vi "HMI.vi"() -> ()   [LabVIEW 2018]
uses:
  <vilib>/Platform/TimedLoop/XDataNode/timing_clust.ctl
  <vilib>/Platform/TimedLoop/XDataNode/nitl_modes.ctl
  <vilib>/Platform/TimedLoop/XDataNode/wakeup.ctl
  <vilib>/Instr/_visa.llb/VISA Configure Serial Port (Instr).vi
  <vilib>/Utility/file.llb/Write Delimited Spreadsheet (DBL).vi
  <vilib>/platform/TimedLoop/XDataNode/XDataNode.xnode
  <vilib>/Platform/TimedLoop/XDataNode/XDNodeRunTimeDep.lvlib
panel:
  out "Tab Control":enum32{"Monitor", "Variables"}(tab)
  in  "cond_i":dbl caption="Condiciones Iniciales:"
  out "b2":dbl
  out "b1":dbl
  out "a1":dbl
  in  "Sim&TR":bool caption="Simulación"
  in  "theta":dbl
  in  "tao":dbl
  in  "K":dbl
  out "Cuenta regresiva":dbl
  in  "Temporizador (s)":dbl
  in  "STOP":bool
  in  "SAVE":bool
  in  "Log":bool
  in  "Auto":bool caption="Modo de Control"
  in  "T_s":dbl=0.0001 caption="Tiempo de Muestreo" min=0.0001 max=15.0 step=0.1
  out "Error":dbl format="%_6g"
  in  "OP":i32 max=100 step=1
  in  "SP":dbl min=0.0 max=300.0 step=1.0 format="%_6g"
  out "PV":dbl format="%_6g"
  out "PLOT 2":cluster{"Error":dbl, "OP":i32}(graph) caption="Error y Manipulación"
  out "PLOT 1":cluster{"PV":dbl, "SP":dbl}(graph) caption="Variable de Proceso (PV) y Referencia (SP)"
  in  "Puerto":refnum<visa-resource-name>
  out "Sample Count":i32 caption="Count"
  out "Tiempo transcurrido (s)":dbl
  in  "baud rate (115200)":u32=9600
  in  "timeout":u32=10000
  in  "data bits (8)":u16=8 min=5 max=8 step=1
  in  "stop bits":u16(ring)=10 items=["1.0"=10, "1.5"=15, "2.0"=20]
  in  "parity":enum16{"None", "Odd", "Even", "Mark", "Space"}(ring)
  in  "flow control":u16(ring) items=["None", "XON/XOFF", "RTS/CTS", "XON/XOFF & RTS/CTS", "DTR/DSR", "XON/XOFF & DTR/DSR"]
  out "Datos":dbl[][](array[numeric])
  out "OP_byte":u8
  out "error out":errorcluster
  out "Cn1":dbl format="%#_13g"
  out "N":i16
  out "m":dbl
  out "Cn":dbl
  out "Temp":dbl
  out "M":i32[](array[numeric])
  # "Auto"
  # "Manual"
  # "Archivar Datos"
  # "on"
  # "off"
  # "Función de diferencias en tiempo discreto (C_n)"
  # "C_n-1 +"
  # "M_n-1-N +"
  # "M_n-2-N"
  # "Creado por David Díaz Paz y Puente\n22/09/2026"
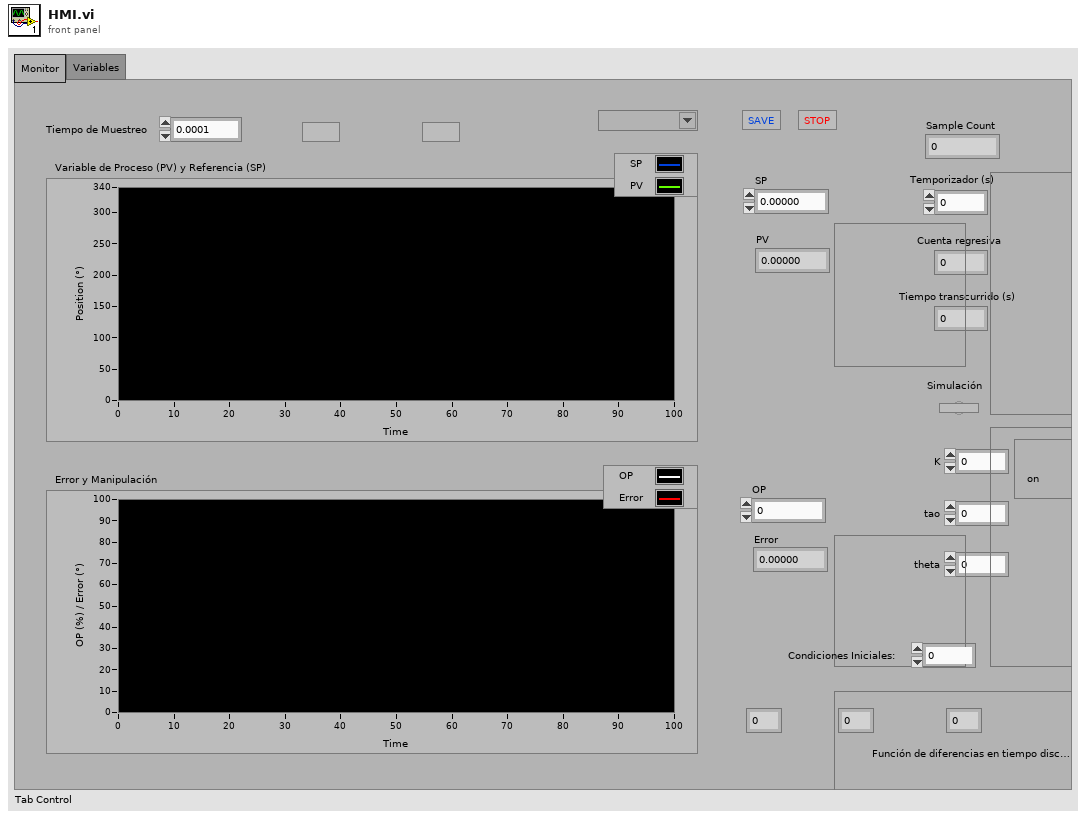
[diagram p1: front panel]
types:
  T1 = typedef "XDNodeRunTimeDep.lvlib/timing_clust.ctl" = cluster{"Expected End [f-1]":u64, "Actual End [f-1]":u64, "Finished Late? [f-1]":bool, "Expected End [i-1]":u64, "Actual End [i-1]":u64, "Finished Late? [i-1]":bool, "Expected Start [i]":u64, "Actual Start [i]":u64, "Expected Start [f]":u64, "Actual Start [f]":u64, "Source Name":string, "Structure Name":string, "Period":i64, "Deadline":i64, "Offset":i64, "Start":i64, "Priority":i32, "Timeout":i32, "Mode":T2, "Wakeup Reason":T3, "Error":errorcluster, "Source Type":string, "Secondary Source Type":string, "Global End Time":u64, "Global Start Time":u64, "Frame Duration":u64, "Iteration Duration":u64, "Assigned CPU":i32, "I/O Scan Engine Mode":u32}
  T2 = typedef "XDNodeRunTimeDep.lvlib/nitl_modes.ctl" = enum32{"No Change", "Process missed periods, maintain original phase", "Discard missed periods, maintain original phase", "Process missed periods, ignore original phase", "Discard missed periods, ignore original phase"}
  T3 = typedef "XDNodeRunTimeDep.lvlib/wakeup.ctl" = enum32{"Normal", "Aborted", "Asynchronous wakeup", "Timing source error", "Timed loop error", "Timeout"}
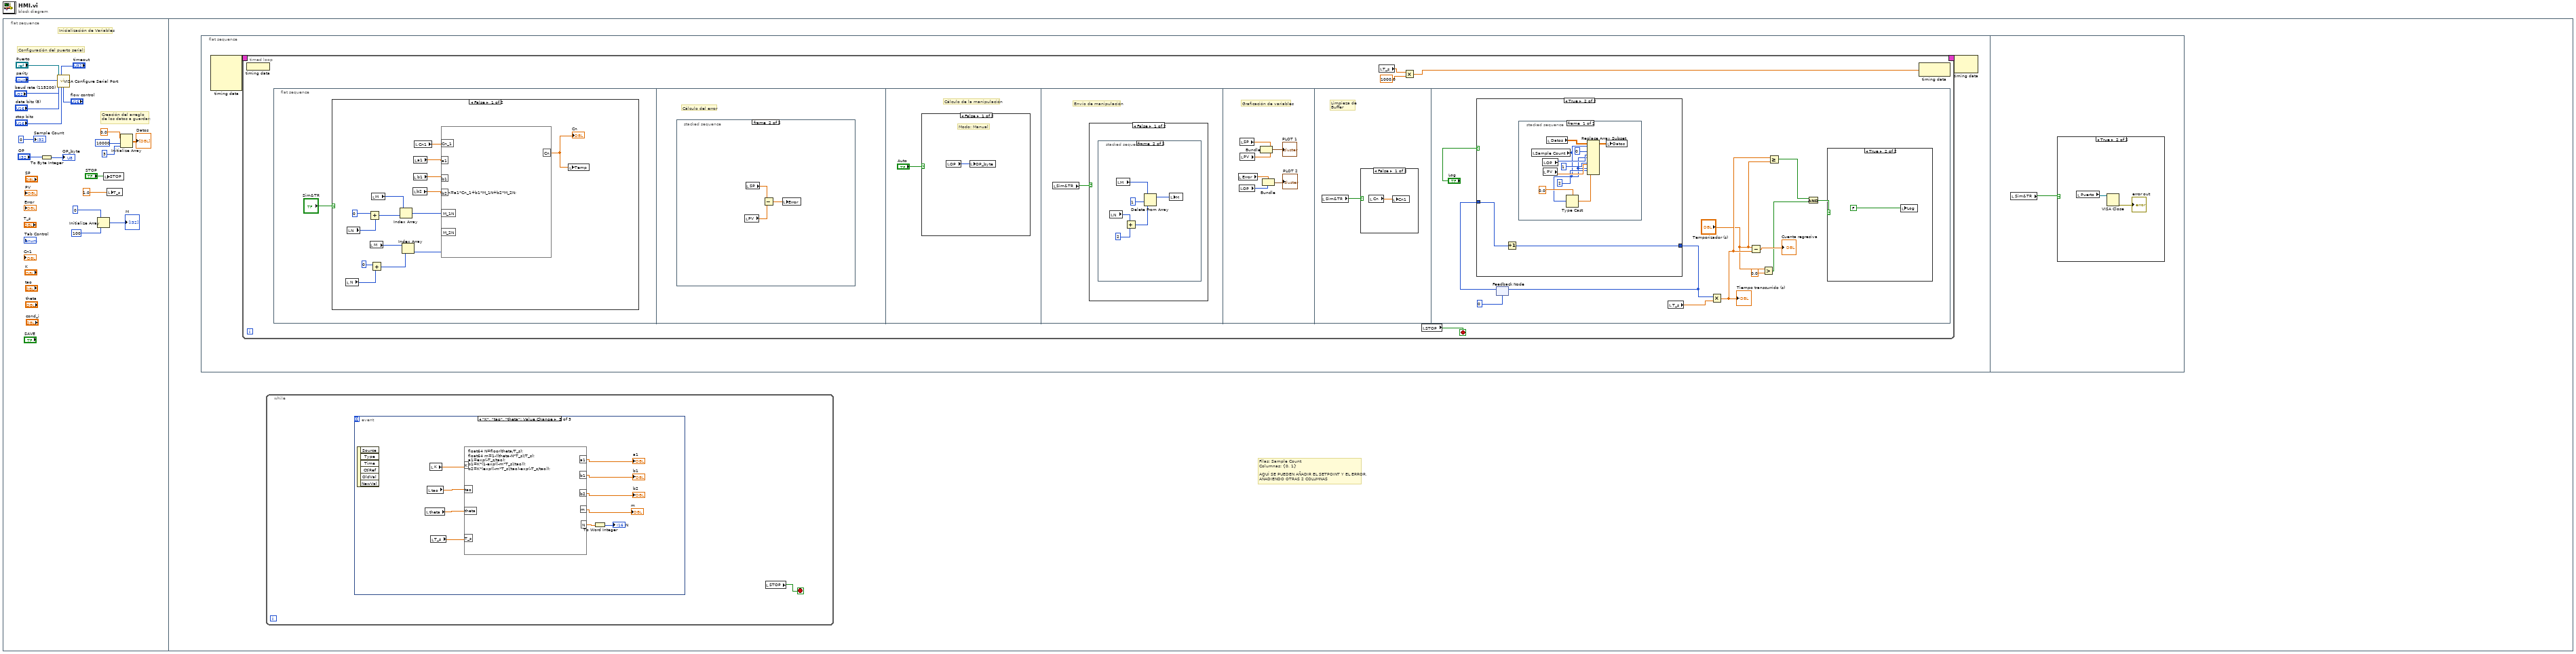
[diagram p0: block diagram]
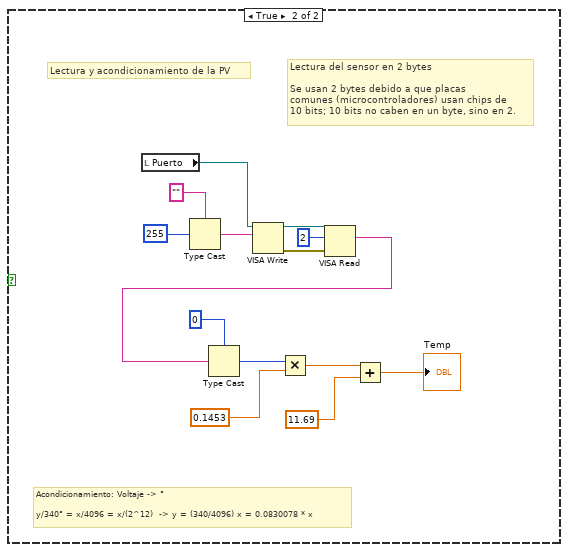
[diagram p2: hidden frame]
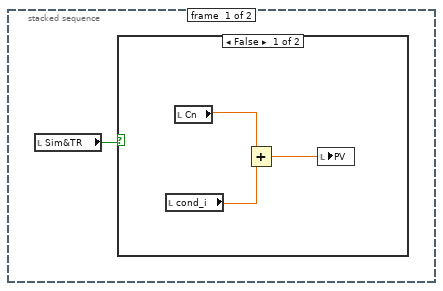
[diagram p3: hidden frame]
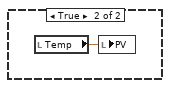
[diagram p4: hidden frame]
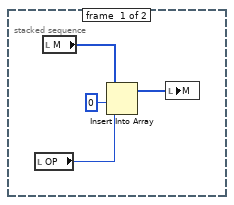
[diagram p6: hidden frame]
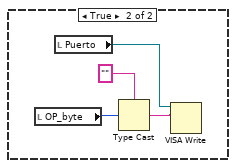
[diagram p7: hidden frame]
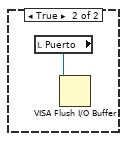
[diagram p8: hidden frame]
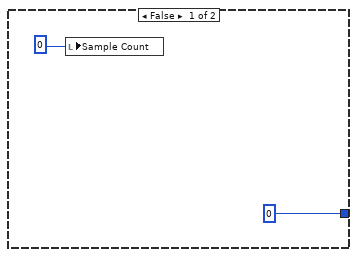
[diagram p10: hidden frame]
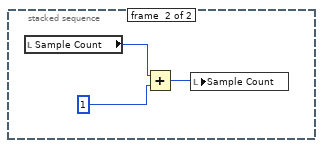
[diagram p11: hidden frame]
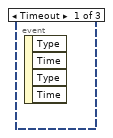
[diagram p13: hidden frame]
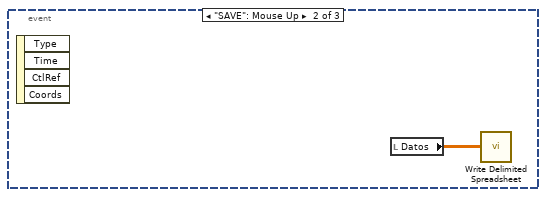
[diagram p14: hidden frame]
diagram:
  n1 = flat-sequence {
    frame #0 {
      # "Creación del arreglo\nde los datos a guardar:"
      # "Configuración del puerto serial:"
      # "Inicialización de Variables"
      n2 = To Byte Integer(number="OP") -> (8bit integer=→"OP_byte":i8)
      n3 = call-poly "VISA Configure Serial Port"("VISA resource name"="Puerto", "timeout (10sec)"="timeout", "baud rate (9600)"="baud rate (115200)", "data bits (8)"="data bits (8)", "parity (0:none)"="parity", "stop bits (10: 1 bit)"="stop bits", "flow control (0:none)"="flow control") -> ()  [unwired: 7 in, 2 out]
      n4 = Initialize Array(0, 100) -> (→"M":i32[])
      n5 = local write "STOP"("STOP") -> ()
      n6 = local write "T_s"(1.0) -> ()
      n7 = Initialize Array(0.0 ("element"), 10000 ("dimension size"), 3 ("dimension size")) -> (→"Datos":dbl[][])
      "Sample Count" <- 0 ("dimension size")
    }
    frame #1 {
      # "Filas: Sample Count\nColumnas: {0, 1}\n\nAQUÍ SE PUEDEN AÑADIR EL SETPOINT Y EL ERROR,\nAÑADIENDO OTRAS 2 COLUMNAS"
      n8 = flat-sequence {
        frame #0 {
          n9 = node-c288() -> (w21:T1)  [unwired: 4 in]
          n10 = timed-loop {
            timing: w21 -> [_]
            timing-out: [_] -> w20
            stop <- w25 stop-if-true
            n11 = node-c288 ("Output Node")() -> ()  [unwired: 1 in]
            n12 = flat-sequence {
              frame #0 {
                n13 = case shown="False" "Sim&TR" {
                  frame False {
                    n14 = local read "N"() -> (w29:i16)
                    n15 = local read "N"() -> (w35:i16)
                    n16 = Add(x=0, y=w35) -> (x+y=w34:i32)
                    n17 = local read "M"() -> (w31:i32[])
                    n18 = Add(x=0, y=w29) -> (x+y=w28:i32)
                    n19 = local read "M"() -> (w33:i32[])
                    n20 = Index Array(array=w33, index=w34) -> (element=w32:i32)
                    n21 = Index Array(array=w31, index=w28) -> (element=w27:i32)
                    n22 = local read "b2"() -> (w40:dbl)
                    n23 = local read "b1"() -> (w39:dbl)
                    n24 = local read "a1"() -> (w38:dbl)
                    n25 = local read "Cn1"() -> (w41:dbl)
                    n26 = formula code="Cn=a1*Cn_1+b1*M_1N+b2*M_2N;"("Cn_1"=w41, "a1"=w38, "b1"=w39, "b2"=w40, "M_1N"=w32, "M_2N"=w27) -> ("Cn"=w37:dbl)
                    "Cn" <- w37
                    n27 = local write "Temp"(w37) -> ()
                  }
                  frame True {
                    # "Acondicionamiento: Voltaje -> °\n\ny/340° = x/4096 = x/(2^12)  -> y = (340/4096) x = 0.0830078 * x"
                    # "Lectura del sensor en 2 bytes\n\nSe usan 2 bytes debido a que placas \ncomunes (microcontroladores) usan chips de\n10 bits; 10 bits no caben en un byte, sino en 2."
                    # "Lectura y acondicionamiento de la PV"
                    n28 = local read "Puerto"() -> (w52:refnum<visa-resource-name>)
                    n29 = Type Cast(type="", x=u8 255 ("type")) -> (*(type *) &x=w53:string)
                    n30 = VISA Write(VISA resource name=w52, write buffer=w53) -> (VISA resource name out=w51:refnum<visa-resource-name>, error out=w50:errorcluster)  [unwired: 1 in, 1 out]
                    n31 = VISA Read(VISA resource name=w51, byte count=i16 2, error in (no error)=w50) -> (read buffer=w42:string)  [unwired: 3 out]
                    n32 = Type Cast(type=i16 0, x=w42) -> (*(type *) &x=w43:i16)
                    n33 = Multiply(x=w43, y=0.1453) -> (x*y=w45:dbl)
                    n34 = Add(x=w45, y=11.69) -> (x+y=→"Temp":dbl)
                  }
                }
              }
              frame #1 {
                # "Cálculo del error"
                n35 = stacked-sequence {
                  frame #0 {
                    n36 = local read "Sim&TR"() -> (w56:bool)
                    n37 = case shown="False" w56 {
                      frame False {
                        n38 = local read "cond_i"() -> (w57:dbl)
                        n39 = local read "Cn"() -> (w58:dbl)
                        n40 = Add(x=w58, y=w57) -> (x+y=w59:dbl)
                        n41 = local write "PV"(w59) -> ()
                      }
                      frame True {
                        n42 = local read "Temp"() -> (w60:dbl)
                        n43 = local write "PV"(w60) -> ()
                      }
                    }
                  }
                  frame #1 {
                    n44 = local read "PV"() -> (w63:dbl)
                    n45 = local read "SP"() -> (w62:dbl)
                    n46 = Subtract(x=w62, y=w63) -> (x-y=w61:dbl)
                    n47 = local write "Error"(w61) -> ()
                  }
                }
              }
              frame #2 {
                # "Cálculo de la manipulación"
                n48 = case shown="False" "Auto" {
                  frame False {
                    # "Modo: Manual"
                    n49 = local read "OP"() -> (w65:i32)
                    n50 = local write "OP_byte"(w65) -> ()
                  }
                  frame True {
                    # "Modo: Automático"
                  }
                }
              }
              frame #3 {
                # "Envío de manipulación"
                n51 = local read "Sim&TR"() -> (w66:bool)
                n52 = case shown="False" w66 {
                  frame False {
                    n53 = stacked-sequence {
                      frame #0 {
                        n54 = local read "OP"() -> (w68:i32)
                        n55 = local read "M"() -> (w70:i32[])
                        n56 = Insert Into Array(array=w70, index=0, new element=w68) -> (w67:i32[])
                        n57 = local write "M"(w67) -> ()
                      }
                      frame #1 {
                        n58 = local read "N"() -> (w74:i16)
                        n59 = local read "M"() -> (w76:i32[])
                        n60 = Add(x=w74, y=i16 2) -> (x+y=w72:i16)
                        n61 = Delete From Array(array=w76, length=1, index=w72) -> (array with subset deleted=w71:i32[])  [unwired: 1 out]
                        n62 = local write "M"(w71) -> ()
                      }
                    }
                  }
                  frame True {
                    n63 = local read "OP_byte"() -> (w79:u8)
                    n64 = local read "Puerto"() -> (w77:refnum<visa-resource-name>)
                    n65 = Type Cast(type="", x=w79) -> (*(type *) &x=w78:string)
                    n66 = VISA Write(VISA resource name=w77, write buffer=w78) -> ()  [unwired: 1 in, 3 out]
                  }
                }
              }
              frame #4 {
                # "Graficación de variables"
                n67 = local read "Error"() -> (w83:dbl)
                n68 = local read "OP"() -> (w82:i32)
                n69 = local read "SP"() -> (w86:dbl)
                n70 = local read "PV"() -> (w85:dbl)
                n71 = Bundle("SP"=w86, "PV"=w85) -> (→"PLOT 1":cluster{"SP":dbl, "PV":dbl})  [unwired: 1 in]
                n72 = Bundle("Error"=w83, "OP"=w82) -> (→"PLOT 2":cluster{"Error":dbl, "OP":i32})  [unwired: 1 in]
              }
              frame #5 {
                # "Limpieza de\nBuffer"
                n73 = local read "Sim&TR"() -> (w87:bool)
                n74 = case shown="False" w87 {
                  frame False {
                    n75 = local read "Cn"() -> (w88:dbl)
                    n76 = local write "Cn1"(w88) -> ()
                  }
                  frame True {
                    n77 = local read "Puerto"() -> (w89:refnum<visa-resource-name>)
                    n78 = VISA Flush I/O Buffer(VISA resource name=w89) -> ()  [unwired: 2 in, 2 out]
                  }
                }
              }
              frame #6 {
                n79 = feedback #1(0) -> (w99:i32)
                n80 = case shown="True" "Log" {
                  tunnel: w99 -> [_ w106]
                  tunnel: [0 w105] -> w98
                  frame False {
                    n81 = local write "Sample Count"(0) -> ()
                  }
                  frame True {
                    n82 = Increment(x=w106) -> (x+1=w105:i32)
                    n83 = stacked-sequence {
                      frame #0 {
                        n84 = local read "Sample Count"() -> (w108:i32)
                        n85 = local read "OP"() -> (w114:i32)
                        n86 = local read "PV"() -> (w112:dbl)
                        n87 = local read "Datos"() -> (w116:dbl[][])
                        n88 = Type Cast(type=0.0 ("y"), x=w108) -> (*(type *) &x=w107:dbl)
                        n89 = Replace Array Subset(array=w116, new element #1=w114, index (row) #1=w108, index (col) #1=0, new element #2=w112, index (row) #2=w108, index (col) #2=1, new element #3=w107, index (row) #3=w108, index (col) #3=2) -> (w111:dbl[][])
                        n90 = local write "Datos"(w111) -> ()
                      }
                      frame #1 {
                        n91 = local read "Sample Count"() -> (w117:i32)
                        n92 = Add(x=w117, y=1) -> (x+y=w119:i32)
                        n93 = local write "Sample Count"(w119) -> ()
                      }
                    }
                  }
                }
                n94 = feedback-in #1(w98) -> ()
                n95 = local read "T_s"() -> (w97:dbl)
                n96 = Multiply(x=w98, y=w97) -> (x*y=w95:dbl)
                "Tiempo transcurrido (s)" <- w95
                n97 = Subtract(x="Temporizador (s)", y=w95) -> (x-y=→"Cuenta regresiva":dbl)
                n98 = Greater?(x="Temporizador (s)", y=0.0) -> (0:w91:bool)
                n99 = Greater Or Equal?(x=w95, y="Temporizador (s)") -> (x >= y?=w92:bool)
                n100 = And(x=w92, y=w91) -> (x .and. y?=w90:bool)
                n101 = case shown="True" w90 {
                  frame False {
                  }
                  frame True {
                    n102 = local write "Log"(FALSE) -> ()
                  }
                }
              }
            }
            n103 = local read "T_s"() -> (w24:dbl)
            n104 = Multiply(x=w24, y=1000.0) -> (x*y=w22:dbl)
            n105 = local read "STOP"() -> (w25:bool)
            n106 = node-c288(w22) -> ()  [unwired: 1 out]
          }
          n107 = node-c288(w20) -> ()  [unwired: 1 out]
        }
        frame #1 {
          n108 = local read "Sim&TR"() -> (w126:bool)
          n109 = case shown="True" w126 {
            frame False {
            }
            frame True {
              n110 = local read "Puerto"() -> (w127:refnum<visa-resource-name>)
              n111 = VISA Close(VISA resource name=w127) -> (error out=→"error out":errorcluster)  [unwired: 1 in]
            }
          }
        }
      }
      n112 = while {
        stop <- w129 stop-if-true
        n113 = event shown="[2] \"K\", \"tao\", \"theta\": Value Change" {
          selector: _ -> [_ _ _]
          dyn-events: _ -> [_ _ _]
          timeout: _ -> [_ _ _]
          event Timeout {
            n114 = event-data() -> ()  [unwired: 1 in, 4 out]
          }
          event "SAVE": Mouse Up {
            n115 = event-data() -> ()  [unwired: 1 in, 4 out]
            n116 = local read "Datos"() -> (w130:dbl[][])
            n117 = call-poly <vilib>:"Write Delimited Spreadsheet.vi"("2D data"=w130) -> ()  [unwired: 13 in, 2 out]
          }
          event "K", "tao", "theta": Value Change {
            n118 = event-data() -> ()  [unwired: 1 in, 6 out]
            n119 = local read "theta"() -> (w138:dbl)
            n120 = local read "tao"() -> (w139:dbl)
            n121 = local read "K"() -> (w140:dbl)
            n122 = local read "T_s"() -> (w137:dbl)
            n123 = formula code="float64 N=floor(theta/T_s);\nfloat64 m=1-((theta-N*T_s)/T_s);\na1=exp(-T_s/tao);\nb1=K*(1-exp((-m*T_s)/tao));\nb2=K*(exp((-m*T_s)/tao)-exp(-T_s/tao));"("K"=w140, "theta"=w138, "tao"=w139, "T_s"=w137) -> ("a1"=→"a1":dbl, "b1"=→"b1":dbl, "b2"=→"b2":dbl, "m"=→"m":dbl, "N"=w136:dbl)
            n124 = To Word Integer(number=w136) -> (16bit integer=→"N":i16)
          }
        }
        n125 = local read "STOP"() -> (w129:bool)
      }
    }
  }
